vi "Actor Core.vi"(8 "error in":errorcluster, 11 "HamamatsuFluor in":refnum<class "HamamatsuFluor.lvclass">) -> (0 "error out":errorcluster, 3 "Actor out":refnum<class "Actor.lvclass">)   [LabVIEW 2020, in "DAQ Timed SPIM.lvlib" / "HamamatsuFluor_v2.lvlib" / "HamamatsuFluor.lvclass"]
doc: "(<B>Filename</B>: Actor Framework.lvlib:Actor.lvclass:Actor Core.vi)\n\nReceives messages to the actor, reacts to them, and initiates any error handling that may shut the actor down.\n\nDescendant classes may override this VI to append parallel tasks for the actor to complete while it handles messages. Overrides use the Call Parent Class Method node."
uses:
  HamamatsuFluor.lvclass
  <vilib>/ActorFramework/Actor/Actor.lvclass
  HamamatsuFluor.lvclass/HamamatsuFluor.ctl
  Abstract DAQ Triggered Actor/Abstract DAQ Triggered Actor.lvclass
  WIN Memory Map.llb/WIN MMAP.lvlib
panel:
  out "Buffer Memory Handle":u64
  out "Buffer Start Pointer":u64
  out "Frame Count":i32
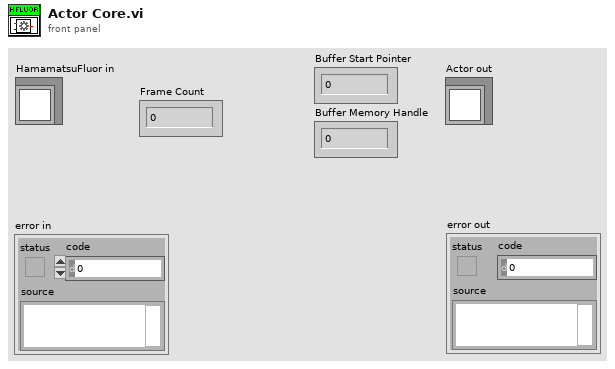
[diagram p1: front panel]
types:
  T1 = enum16{"big-endian, network order", "native, host order", "little-endian"}
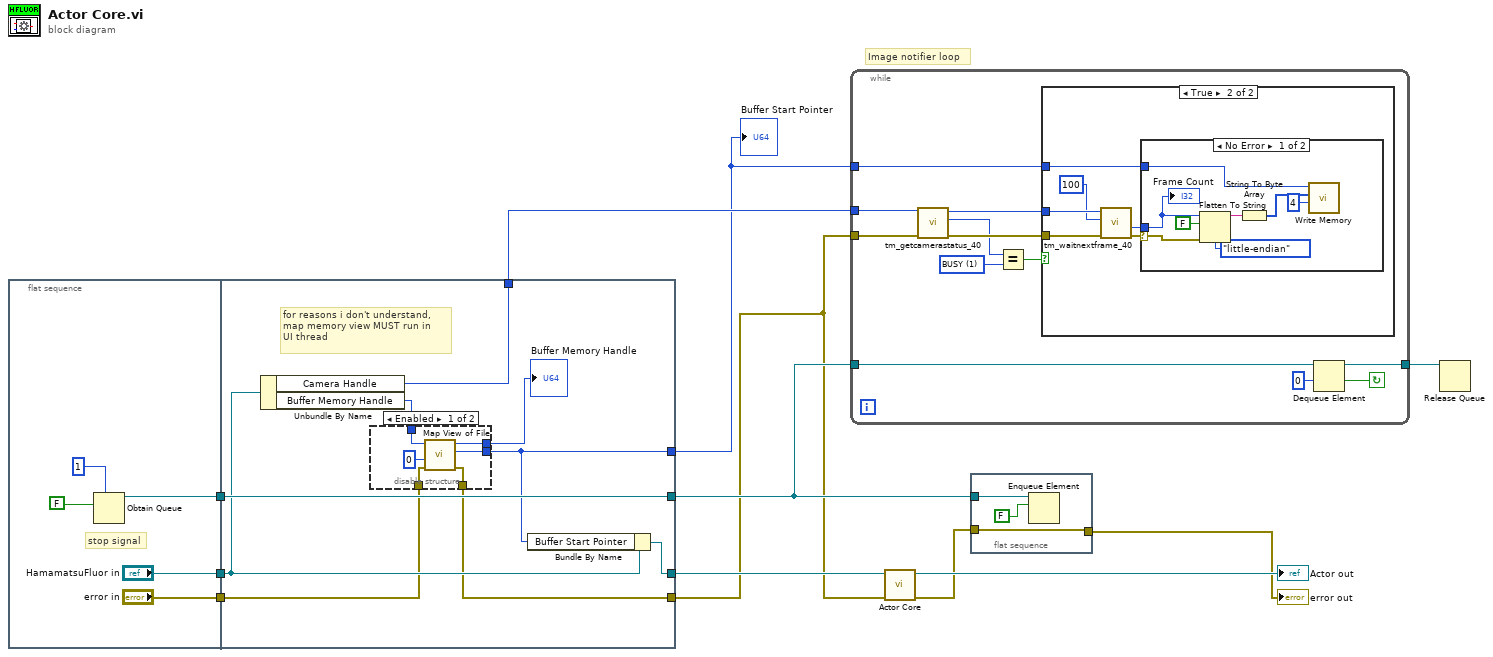
[diagram p0: block diagram]
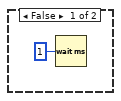
[diagram p3: hidden frame]
diagram:
  # "Image notifier loop"
  n1 = flat-sequence {
    tunnel: ["error in"] -> w5
    tunnel: ["HamamatsuFluor in"] -> w4
    tunnel: [w14] -> w3
    tunnel: [w26] -> w9
    tunnel: [w23] -> w10
    tunnel: [w20] -> w6
    tunnel: w5 -> [w21]
    tunnel: w4 -> [w24]
    tunnel: w3 -> [w26]
    tunnel: [w25] -> w2
    tunnel: [w18] -> w1
    frame #0 {
      # "stop signal"
      n2 = Obtain Queue(max queue size (-1, unlimited)=1, element data type=FALSE) -> (queue out=w14:refnum<queue>)  [unwired: 3 in, 2 out]
    }
    frame #1 {
      # "for reasons i don't understand,\nmap memory view MUST run in\nUI thread"
      n3 = Unbundle By Name(w24) -> ("Camera Handle"=w25:u32, "Buffer Memory Handle"=w22:u64)
      n4 = disable-structure shown="Enabled" {
        disable-tunnel: w22 -> [w32 w34]
        disable-tunnel: w21 -> [w30 w33]
        disable-tunnel: [w29 w33] -> w20
        disable-tunnel: [w28 w34] -> w19
        disable-tunnel: [w27 _] -> w18
        frame Enabled {
          n5 = call "Map View of File.vi"("error in (no error)"=w30, "offset"=u32 0, "handle"=w32) -> ("error out"=w29:errorcluster, "startAddress"=w27:u64, "handle out"=w28:u64)  [unwired: 6 in]
        }
        frame Disabled {
        }
      }
      "Buffer Memory Handle" <- w19
      n6 = Bundle By Name(cluster=w24, "Buffer Start Pointer"=w18) -> (w23:refnum<class "HamamatsuFluor.lvclass">)
    }
  }
  n7 = while {
    tunnel: w2 -> [w46]
    tunnel: w6 -> [w40]
    tunnel: w9 -> [w39]
    tunnel: [w37] -> w7
    tunnel: w1 -> [w35]
    stop <- w36 continue-if-true
    w45 = 1 items=["ERROR", "BUSY", "READY", "STABLE", "UNSTABLE"] ("Status")
    n8 = call <userlib>:"tm_getcamerastatus_40.vi"("error in (no error)"=w40, "Handle in"=w46) -> ("error out"=w42:errorcluster, "Status"=w41:i32, "Handle out"=w43:u32)  [unwired: 7 in]
    n9 = Equal?(x=w41, y=w45) -> (x = y?=w44:bool)
    n10 = case shown="True" w44 {
      tunnel: w43 -> [_ w53]
      tunnel: w42 -> [_ w52]
      tunnel: w35 -> [_ w48]
      frame False {
        n11 = Wait (ms)(milliseconds to wait=u32 1) -> ()  [unwired: 1 out]
      }
      frame True {
        n12 = call <userlib>:"tm_waitnextframe_40.vi"("error in (no error)"=w52, "Timeout"=100, "Handle in"=w53) -> ("error out"=w51:errorcluster, "Frame Count"=w49:i32)  [unwired: 5 in, 2 out]
        n13 = case shown="No Error" w51 {
          selector: w51 -> [w60 _]
          tunnel: w49 -> [w59 _]
          tunnel: w48 -> [w61 _]
          frame No Error {
            n14 = Flatten To String(anything=w59, prepend array or string size? (T)=FALSE, byte order (0:big-endian, network order)=T1."little-endian", error in (no error)=w60) -> (data string=w58:string)  [unwired: 2 out]
            n15 = String To Byte Array(string=w58) -> (unsigned byte array=w57:u8[])
            n16 = call "Write Memory.vi"("offset"=u32 4, "data"=w57, "startAddress"=w61) -> ()  [unwired: 7 in, 2 out]
            "Frame Count" <- w59
          }
          frame Error {
          }
        }
      }
    }
    n17 = Dequeue Element(queue=w39, timeout in ms (-1)=0) -> (queue out=w37:refnum<queue>, timed out?=w36:bool)  [unwired: 1 in, 2 out]
  }
  n18 = call-parent "Actor Core.vi"("error in"=w6, "Actor in"=w10) -> ("error out"=w11:errorcluster, "Actor out"=→"Actor out":refnum<class "Actor.lvclass">)  [unwired: 8 in]
  n19 = flat-sequence {
    tunnel: w11 -> [w62]
    tunnel: w9 -> [w64]
    tunnel: [w62] -> w8
    frame #0 {
      n20 = Enqueue Element(queue=w64, element=FALSE) -> ()  [unwired: 2 in, 3 out]
    }
  }
  n21 = Release Queue(queue=w7) -> ()  [unwired: 2 in, 3 out]
  "error out" <- w8
  "Buffer Start Pointer" <- w1
